vi "配置动效风格.vi"(5 "已初始化":bool, 7 "已隐藏不需要的遮罩层":bool, 8 "error in (no error)":errorcluster caption="错误输入（无错误）", 10 "动效风格":enum16{"风格一", "风格二", "风格三", "风格四"}(ring), 11 "遮罩层引用":refnum<vi>[](array[refnum])) -> (0 "error out":errorcluster caption="错误输出", 2 "动效2引用":refnum<vi>, 3 "动效1引用":refnum<vi>)   [LabVIEW 2025, in "XButton.lvlib" / "button3.xctl"]
uses:
  button3.xctl
  <vilib>/Utility/miscctls.llb/LVPositionTypeDef.ctl
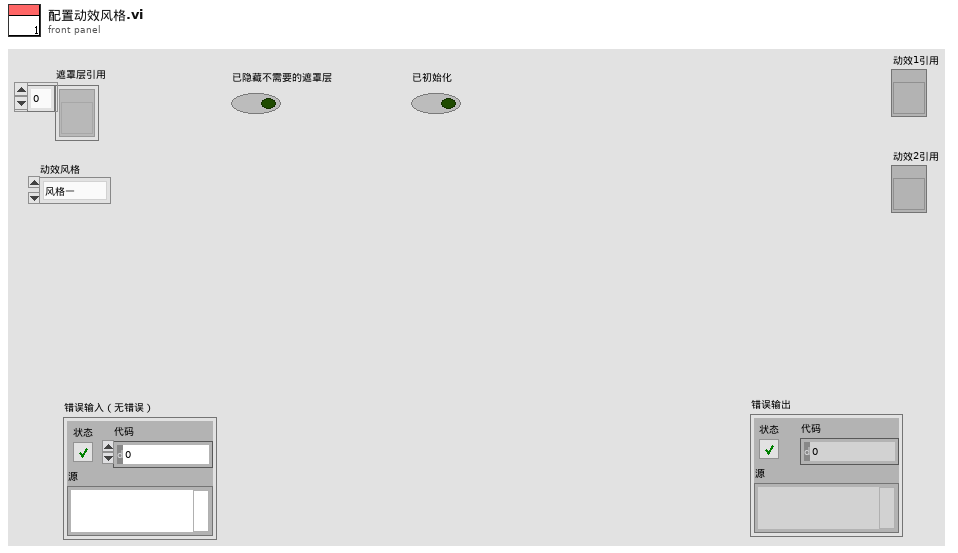
[diagram p1: front panel]
types:
  T1 = typedef "LVPositionTypeDef.ctl" = cluster{"Left":i32, "Top":i32}
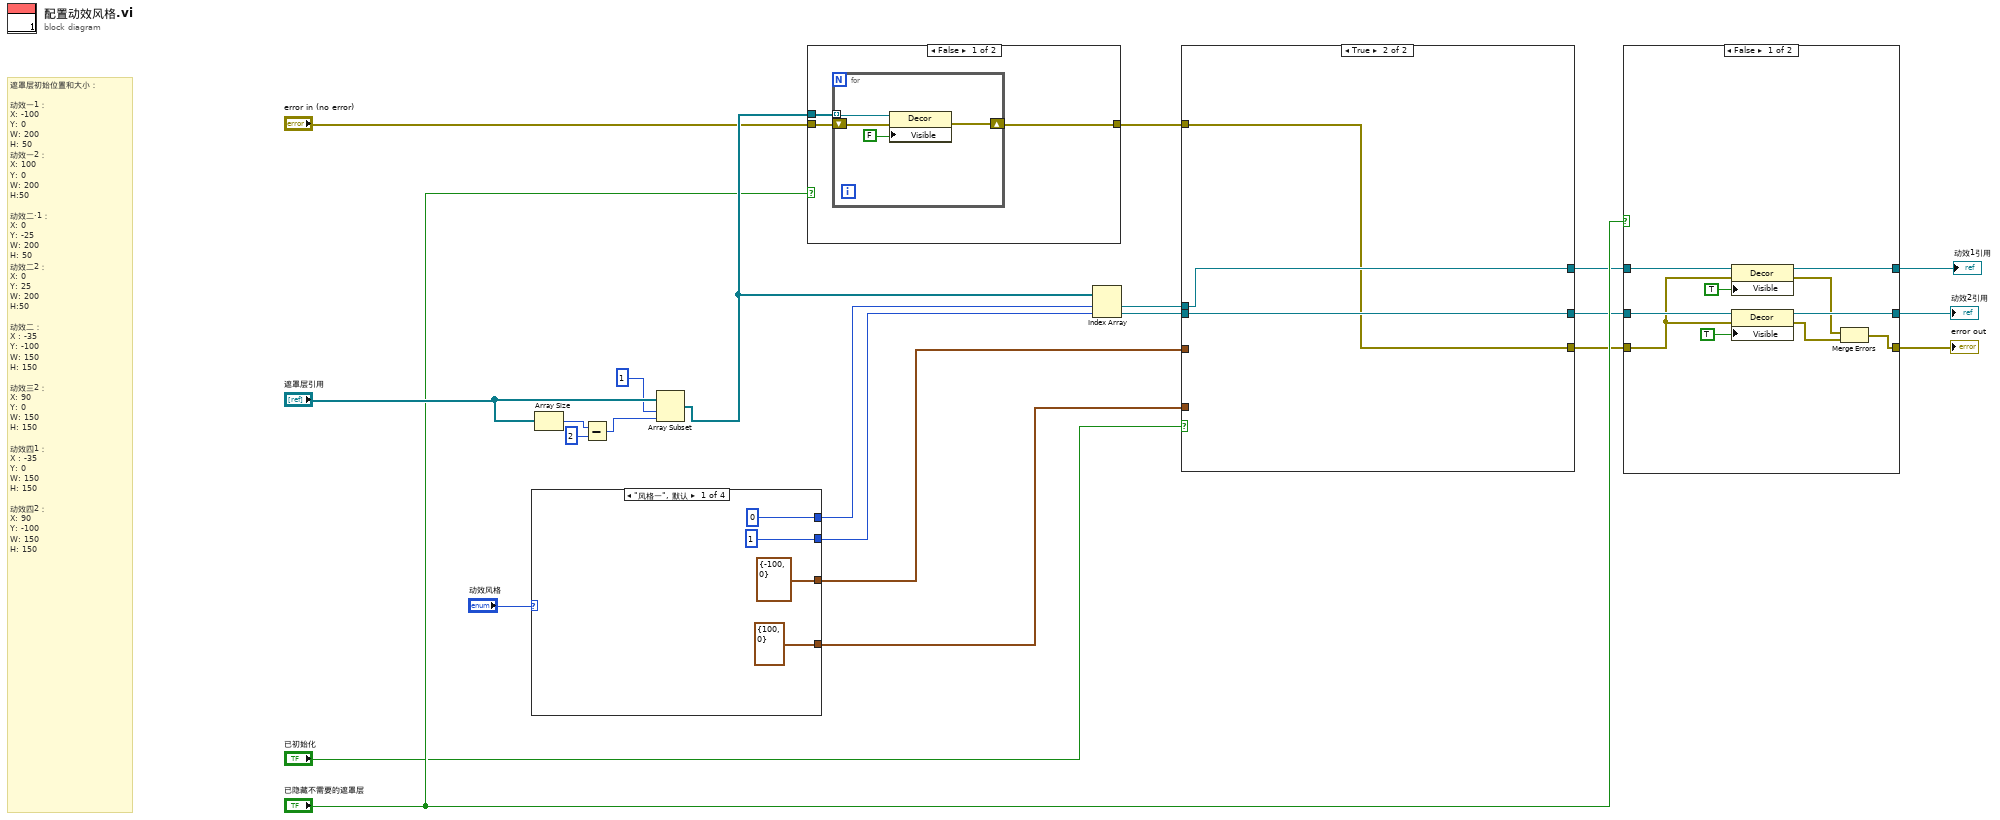
[diagram p0: block diagram]
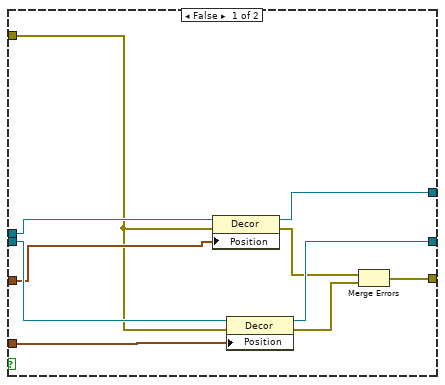
[diagram p2: hidden frame]
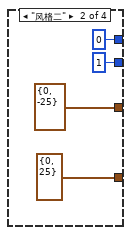
[diagram p5: hidden frame]
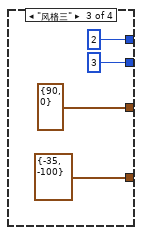
[diagram p6: hidden frame]
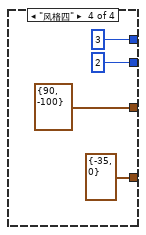
[diagram p7: hidden frame]
diagram:
  # "遮罩层初始位置和大小：\n\n动效一1：\nX: -100\nY: 0\nW: 200\nH: 50\n动效一2：\nX: 100\nY: 0\nW: 200\nH:50\n\n动效二·1：\nX: 0\nY: -25\nW: 200\nH: 50\n动效二2：\nX: 0\nY: 25\nW: 200\nH:50\n\n动效二：\nX : -35\nY: -100\nW: 150\nH: 150\n\n动效三2：\nX: 90\nY: 0\nW: 150\nH: 150\n\n动效四1：\nX : -35\nY: 0\nW: 150\nH: 150\n\n动效四2：\nX: 90\nY: -100\nW: 150\nH: 150"
  n1 = case shown="\"风格一\", 默认" "动效风格" {
    tunnel: [0 0 2 3] -> w17
    tunnel: [1 1 3 2] -> w16
    tunnel: [T1 {"Left"=-100, "Top"=0} ("位置") T1 {"Left"=0, "Top"=-25} ("位置") T1 {"Left"=90, "Top"=0} ("位置") T1 {"Left"=90, "Top"=-100} ("位置")] -> w5
    tunnel: [T1 {"Left"=100, "Top"=0} ("位置") T1 {"Left"=0, "Top"=25} ("位置") T1 {"Left"=-35, "Top"=-100} ("位置") T1 {"Left"=-35, "Top"=0} ("位置")] -> w4
    frame "风格一", Default {
    }
    frame "风格二" {
    }
    frame "风格三" {
    }
    frame "风格四" {
    }
  }
  n2 = Array Size(array="遮罩层引用") -> (size(s)=w23:i32)
  n3 = Subtract(x=w23, y=2) -> (x-y=w19:i32)
  n4 = Array Subset(array="遮罩层引用", index=1 ("索引"), length=w19) -> (w13:refnum<vi>[])
  n5 = case shown="False" "已隐藏不需要的遮罩层" {
    tunnel: w13 -> [w42 _]
    tunnel: "error in (no error)" -> [w41 w47]
    tunnel: [w40 w47] -> w3
    frame False {
      n6 = for {
        tunnel: w42 -> [w46] mode=indexing
        shift-right: [w43] -> w40
        shift-left: w41 -> [w44]
        n7 = property class="Decor"(reference=w46, error in=w44, "Visible"=FALSE ("可见")) -> (error out=w43:errorcluster)  [unwired: 1 out]
      }
    }
    frame True {
    }
  }
  n8 = Index Array(array=w13, index #1=w17, index #2=w16) -> (element #1=w9:refnum<vi>, element #2=w8:refnum<vi>)
  n9 = case shown="True" "已初始化" {
    tunnel: w9 -> [w57 w60]
    tunnel: w8 -> [w55 w59]
    tunnel: [w56 w60] -> w7
    tunnel: [w54 w59] -> w6
    tunnel: w5 -> [w53 _]
    tunnel: w4 -> [w52 _]
    tunnel: w3 -> [w51 w58]
    tunnel: [w48 w58] -> w2
    frame False {
      n10 = property class="Decor"(reference=w57, error in=w51, "Position"=w53) -> (reference out=w56:refnum<vi>, error out=w50:errorcluster)
      n11 = property class="Decor"(reference=w55, error in=w51, "Position"=w52) -> (reference out=w54:refnum<vi>, error out=w49:errorcluster)
      n12 = Merge Errors(w50, w49) -> (w48:errorcluster)
    }
    frame True {
    }
  }
  n13 = case shown="False" "已隐藏不需要的遮罩层" {
    tunnel: w7 -> [w70 w73]
    tunnel: [w69 w73] -> w15
    tunnel: [w68 w72] -> w14
    tunnel: w6 -> [w65 w72]
    tunnel: w2 -> [w64 w71]
    tunnel: [w61 w71] -> w1
    frame False {
      n14 = property class="Decor"(reference=w70, error in=w64, "Visible"=TRUE ("可见")) -> (reference out=w69:refnum<vi>, error out=w63:errorcluster)
      n15 = property class="Decor"(reference=w65, error in=w64, "Visible"=TRUE ("可见")) -> (reference out=w68:refnum<vi>, error out=w62:errorcluster)
      n16 = Merge Errors(w63, w62) -> (w61:errorcluster)
    }
    frame True {
    }
  }
  "error out" <- w1
  "动效1引用" <- w15
  "动效2引用" <- w14
